vi "Execute.vi"(8 "error in (no error)":errorcluster, 11 "Node in":refnum<class "bt_Repeater.lvclass">) -> (0 "error out":errorcluster, 1 "Status":T1, 3 "Node out":refnum<class "bt_Repeater.lvclass">)   [LabVIEW 2021, in "BT.lvlib" / "bt_Repeater.lvclass"]
uses:
  bt_Repeater.lvclass
  abs_Node/Status.ctl
  bt_Repeater.lvclass/bt_Repeater.ctl
  Support/Decorator/bt_Decorator.lvclass
  abs_Node/bt_Node.lvclass
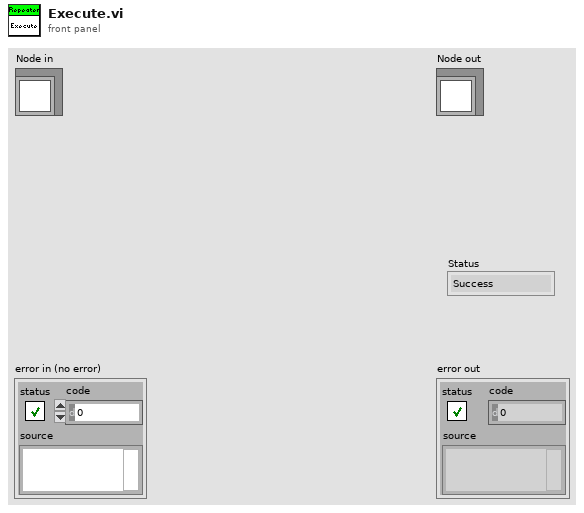
[diagram p1: front panel]
types:
  T1 = typedef "BT.lvlib/bt_Node.lvclass/Status.ctl" = enum16{"Success", "Failure", "Running"}
  T2 = typedef "BT.lvlib/Repeater.lvclass/Finish On - Type.ctl" = enum16{"Success", "Failure", "Never"}
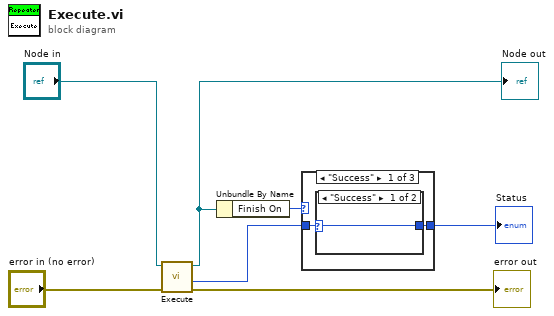
[diagram p0: block diagram]
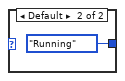
[diagram p2: hidden frame]
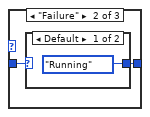
[diagram p3: hidden frame]
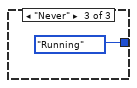
[diagram p5: hidden frame]
diagram:
  n1 = call-parent "Execute.vi"("error in (no error)"="error in (no error)", "Node in"="Node in") -> ("error out"=→"error out":errorcluster, "Status"=w1:T1, "Node out"=w5:refnum<class "bt_Repeater.lvclass">)  [unwired: 7 in]
  "Node out" <- w5
  n2 = Unbundle By Name(w5) -> ("Finish On"=w2:T2)
  n3 = case shown="\"Success\"" w2 {
    tunnel: w1 -> [w8 w12 _]
    tunnel: [w9 w13 Status."Running" ("Status")] -> w4
    frame "Success" {
      n4 = case shown="\"Success\"" w8 {
        selector: w8 -> [w10 _]
        tunnel: [w10 Status."Running" ("Status")] -> w9
        frame "Success" {
        }
        frame Default {
        }
      }
    }
    frame "Failure" {
      n5 = case shown="Default" w12 {
        selector: w12 -> [_ w15]
        tunnel: [Status."Running" ("Status") w15] -> w13
        frame Default {
        }
        frame "Failure" {
        }
      }
    }
    frame "Never" {
    }
  }
  "Status" <- w4
